vi "RemoteVI Fixture Mouse Line.vi"(0 "kind":string, 1 "CtlRef":refnum<vi>, 2 "Coords":cluster{"Horizontal":i32, "Vertical":i32}, 3 "Button":u16, 4 "PlatMods":T1, 5 "error in":errorcluster) -> (14 "line":string, 19 "error out":errorcluster)   [LabVIEW 2020]
doc: "Event-log helper of RemoteVI Fixture.vi. Builds one mouse line of the log: kind TAB label TAB x y button mods LF, where kind is mousedown or mouseup, label is read from the event's control reference, x y are the event's Coords, button its Button and mods the held modifiers as RemoteVI Fixture Mods.vi writes them. Errors of reading the label go to error out."
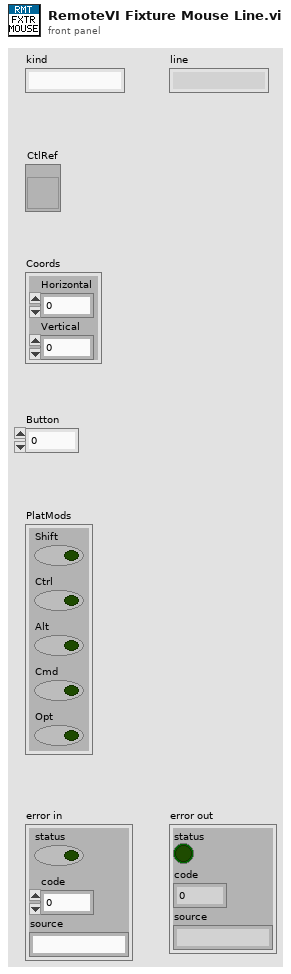
[diagram p1: front panel]
types:
  T1 = cluster{"Shift":bool, "Ctrl":bool, "Alt":bool, "Cmd":bool, "Opt":bool}
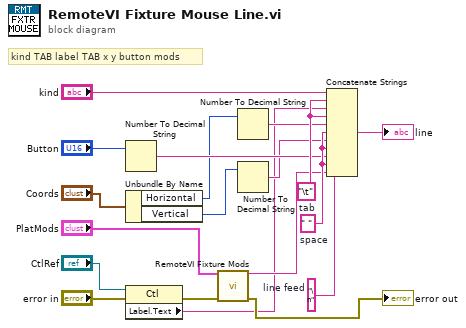
[diagram p0: block diagram]
diagram:
  w18 = "\n"  # line feed
  w17 = " "  # space
  w16 = "\t"  # tab
  # "kind TAB label TAB x y button mods"
  n1 = Number To Decimal String(number="Button") -> (decimal integer string=w13:string)  [unwired: 1 in]
  n2 = Unbundle By Name("Coords") -> ("Horizontal"=w9:i32, "Vertical"=w10:i32)
  n3 = property class="Ctl"(reference="CtlRef", error in="error in") -> (error out=w8:errorcluster, "Label.Text"=w7:string)  [unwired: 1 out]
  n4 = call "RemoteVI Fixture Mods.vi"("PlatMods"="PlatMods", "error in"=w8) -> ("mods"=w14:string, "error out"=→"error out":errorcluster)  [unwired: 12 in]
  n5 = Number To Decimal String(number=w9) -> (decimal integer string=w11:string)  [unwired: 1 in]
  n6 = Number To Decimal String(number=w10) -> (decimal integer string=w12:string)  [unwired: 1 in]
  n7 = Concatenate Strings("kind", w16, w7, w16, w11, w17, w12, w17, w13, w17, w14, w18) -> (→"line":string)
